vi "File Path Extract.vi"(0 "DPE Project File Path":string) -> (11 ".digitdr file path":path, 12 "Timing path name":string, 13 "Level path name":string, 14 "DPE Project Path":path, 15 ".pinmap file path":path, 16 "DPI Instrument Name":string, 17 ".digitiming file path":path, 18 ".digilevels file path":path, 19 ".spec file path":path)   [LabVIEW 2025, in "Digital Pattern Sequencer.lvclass"]
uses:
  Digital Pattern Sequencer.lvclass
  Digital Pattern Sequencer.lvclass/Digital Pattern Sequencer.ctl
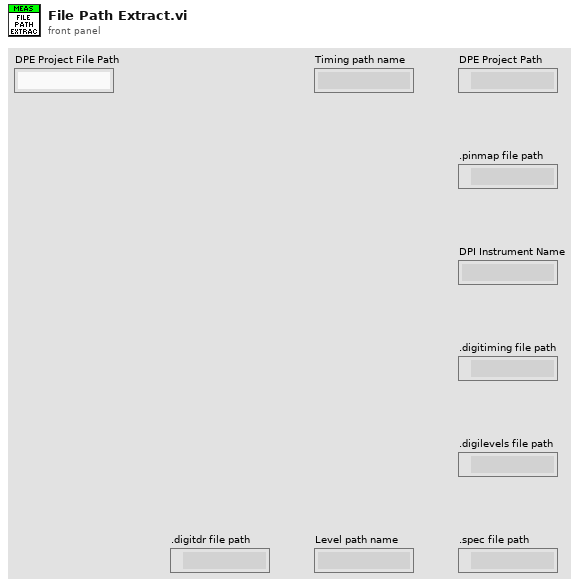
[diagram p1: front panel]
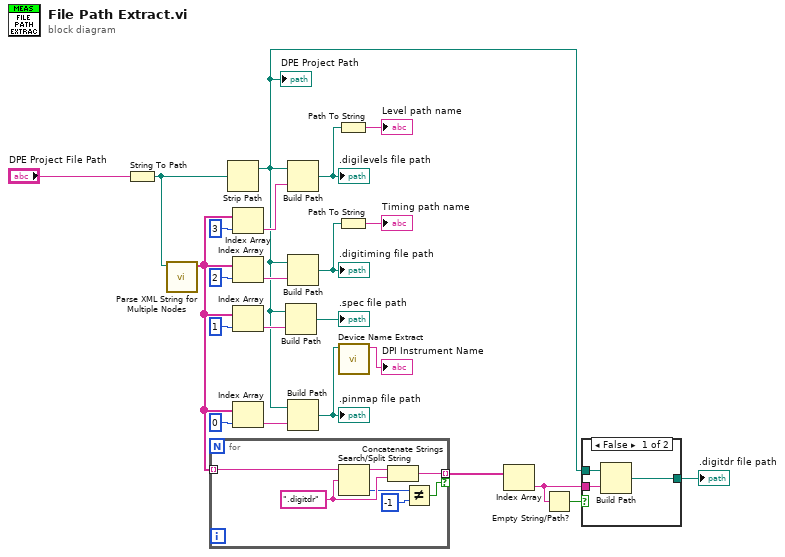
[diagram p0: block diagram]
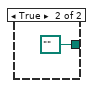
[diagram p2: hidden frame]
diagram:
  n1 = String To Path(string="DPE Project File Path") -> (path=w14:path)
  n2 = call "Parse XML String for Multiple Nodes.vi"("file (use dialog)"=w14) -> ("Array"=w6:string[])  [unwired: 10 in]
  n3 = for {
    tunnel: w6 -> [w30] mode=indexing
    tunnel: [w27] -> w4 mode=indexing if=w24
    w28 = ".digitdr" ("search string/char (-)")
    n4 = Search/Split String(string=w30, search string/char (-)=w28) -> (substring before match=w29:string, offset of match=w26:i32)  [unwired: 1 in, 1 out]
    n5 = Concatenate Strings(w29, w28) -> (w27:string)
    n6 = Not Equal?(x=w26, y=-1) -> (x != y?=w24:bool)
  }
  n7 = Strip Path(path=w14) -> (stripped path=w5:path)  [unwired: 1 out]
  "DPE Project Path" <- w5
  n8 = Index Array(array=w6, index=3) -> (element=w18:string)
  n9 = Index Array(array=w6, index=2) -> (element=w17:string)
  n10 = Index Array(array=w6, index=1) -> (element=w16:string)
  n11 = Index Array(array=w6, index=0) -> (element=w15:string)
  n12 = Build Path(base path=w5, name or relative path=w16) -> (appended path=→".spec file path":path)
  n13 = Build Path(base path=w5, name or relative path=w18) -> (appended path=w9:path)
  ".digilevels file path" <- w9
  n14 = Build Path(base path=w5, name or relative path=w17) -> (appended path=w10:path)
  ".digitiming file path" <- w10
  n15 = Build Path(base path=w5, name or relative path=w15) -> (appended path=w11:path)
  ".pinmap file path" <- w11
  n16 = Path To String(path=w9) -> (string=→"Level path name":string)
  n17 = Path To String(path=w10) -> (string=→"Timing path name":string)
  n18 = call "Device Name Extract.vi"(".pinmap File Path"=w11) -> ("Device Name"=→"DPI Instrument Name":string)  [unwired: 10 in]
  n19 = Index Array(array=w4) -> (element=w2:string)  [unwired: 1 in]
  n20 = Empty String/Path?(string/path=w2) -> (empty?=w3:bool)
  n21 = case shown="False" w3 {
    tunnel: w5 -> [w33 _]
    tunnel: w2 -> [w32 _]
    tunnel: [w31 path "" ("appended path")] -> w1
    frame False {
      n22 = Build Path(base path=w33, name or relative path=w32) -> (appended path=w31:path)
    }
    frame True {
    }
  }
  ".digitdr file path" <- w1
